vi "FuncVI_Sub - VI - finally run VI.vi"(7 "open FP":bool, 8 "error in":errorcluster, 10 "Wait until done":bool, 11 "vi RefNum":refnum<vi>) -> (0 "error out":errorcluster)   [LabVIEW 2021]
doc: "::: CalcExpress Toolkit :::\nCopyright (c) 2000-2026 Konstantin Shifershteyn. All rights reserved."
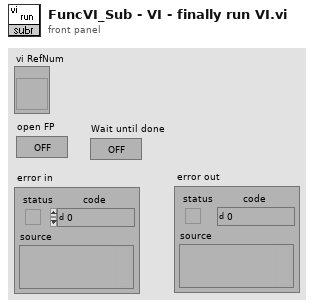
[diagram p1: front panel]
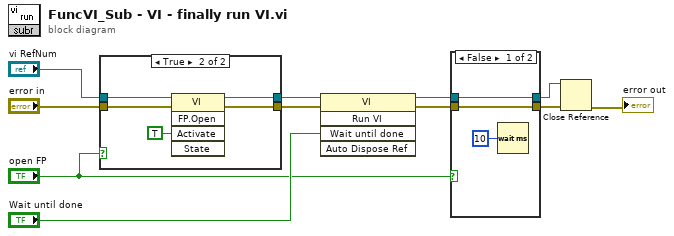
[diagram p0: block diagram]
diagram:
  n1 = case shown="True" "open FP" {
    tunnel: [w12 w15] -> w11
    tunnel: [w13 w17] -> w10
    tunnel: "error in" -> [w12 w16]
    tunnel: "vi RefNum" -> [w13 w18]
    frame False {
    }
    frame True {
      n2 = invoke class="VI" method="FP.Open"(reference=w18, error in=w16, "Activate"=TRUE ("Activate?")) -> (reference out=w17:refnum<vi>, error out=w15:errorcluster)  [unwired: 2 in, 3 out]
    }
  }
  n3 = invoke class="VI" method="Run VI"(reference=w10, error in=w11, "Wait until done"="Wait until done") -> (reference out=w4:refnum<vi>, error out=w5:errorcluster)  [unwired: 2 in, 3 out]
  n4 = case shown="False" "open FP" {
    tunnel: w5 -> [w21 w22]
    tunnel: [w21 w22] -> w3
    tunnel: [w20 w23] -> w2
    tunnel: w4 -> [w20 w23]
    frame False {
      n5 = Wait (ms)(milliseconds to wait=u32 10) -> ()  [unwired: 1 out]
    }
    frame True {
    }
  }
  n6 = Close Reference(reference=w2, error in (no error)=w3) -> (error out=→"error out":errorcluster)
